vi "VIH UI - Path Indication (with Default).vi"(9 "Ena Empty Path":bool, 11 "Path":path) -> (0 "Custom":bool, 1 "Disable":u8, 3 "Path out":path)   [LabVIEW 2014]
doc: "::: VI Helpeks :::\nCopyright (c) 2000-2026 Konstantin Shifershteyn. All rights reserved."
panel:
  # "VI Helpeks\nCopyright (c) 2012-2026 Konstantin Shifershteyn"
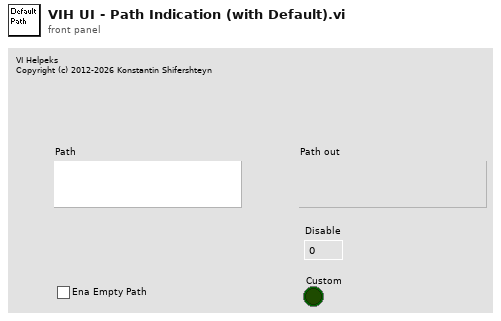
[diagram p1: front panel]
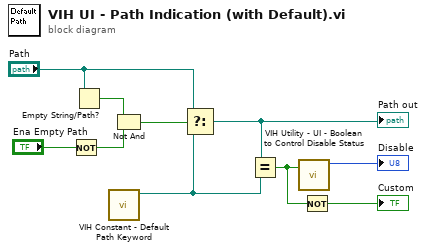
[diagram p0: block diagram]
diagram:
  n1 = Not(x="Ena Empty Path") -> (.not. x?=w6:bool)
  n2 = Empty String/Path?(string/path="Path") -> (empty?=w5:bool)
  n3 = call "VIH Constant - Default Path Keyword.vi"() -> ("<default> path"=w1:path)  [unwired: 11 in]
  n4 = Not And(1:w6, 2:w5) -> (0:w4:bool)
  n5 = Select(t="Path", s=w4, f=w1) -> (s? t:f=w2:path)
  "Path out" <- w2
  n6 = Equal?(x=w2, y=w1) -> (x = y?=w10:bool)
  n7 = call "VIH Utility - UI - Boolean to Control Disable Status.vi"("Status in"=w10) -> ("Control Disable if True"=→"Disable":u8)  [unwired: 3 in, 1 out]
  n8 = Not(x=w10) -> (.not. x?=→"Custom":bool)
